vi "Day Total Entries.vi"(8 "error in":errorcluster, 10 "Day":timestamp, 11 "Time Entry Store in":refnum<class "Time Entry Store.lvclass">) -> (0 "error out":errorcluster, 2 "Total Entries":T1, 3 "Time Entry Store out":refnum<class "Time Entry Store.lvclass">)   [LabVIEW 2026]
doc: "Collects the time entries that count towards the total of one local calendar day, for Day Total.vi. Call it once when a day is loaded; it reads the store.\n\nReturns every entry that starts on the day (as the Time Entry Store's Read Entries for Day gives them) plus every entry that started on the previous day and either ends after the day's local midnight or is still running (End Time 0). The previous day is read through the store too, so the store picks the month files (the previous day may be in the previous month). Day starts are calendar-correct local midnights (Increment_Decrement by one Day.vi), so daylight saving days are handled. Entries are de-duplicated by ID and ordered by Start Time.\n\nInputs: Time Entry Store in; Day (any time within the local day); error in.\nOutputs: Time Entry Store out; Total Entries; error out.\n\nGenerated by: Claude"
uses:
  Storage/Time Entry Store/Time Entry Store.lvclass
  Storage/Rows/Time Entry List.ctl
  Storage/Rows/Time Entry.ctl
  Utilities/Time Management/ENUM-Inc_Dec.ctl
  Utilities/Time Management/Time Management.lvlib
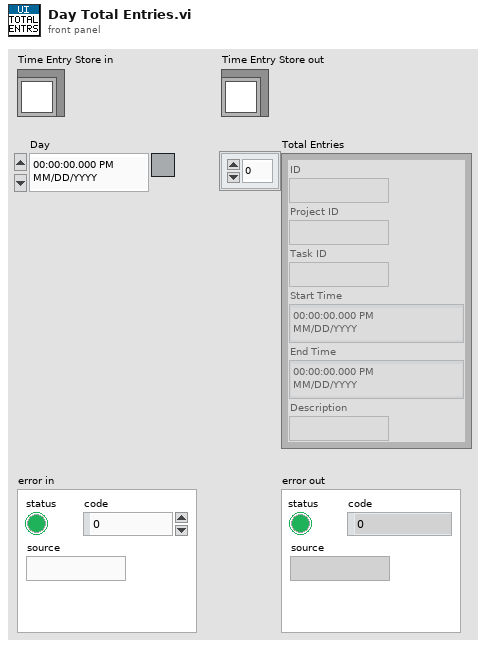
[diagram p1: front panel]
types:
  T1 = typedef "Time Entry List.ctl" = T2[]
  T2 = typedef "Time Entry.ctl" = cluster{"ID":string, "Project ID":string, "Task ID":string, "Start Time":timestamp, "End Time":timestamp, "Description":string}
  T3 = typedef "ENUM-Inc_Dec.ctl" = enum16{"NO CHANGE", "Increment", "Decrement"}
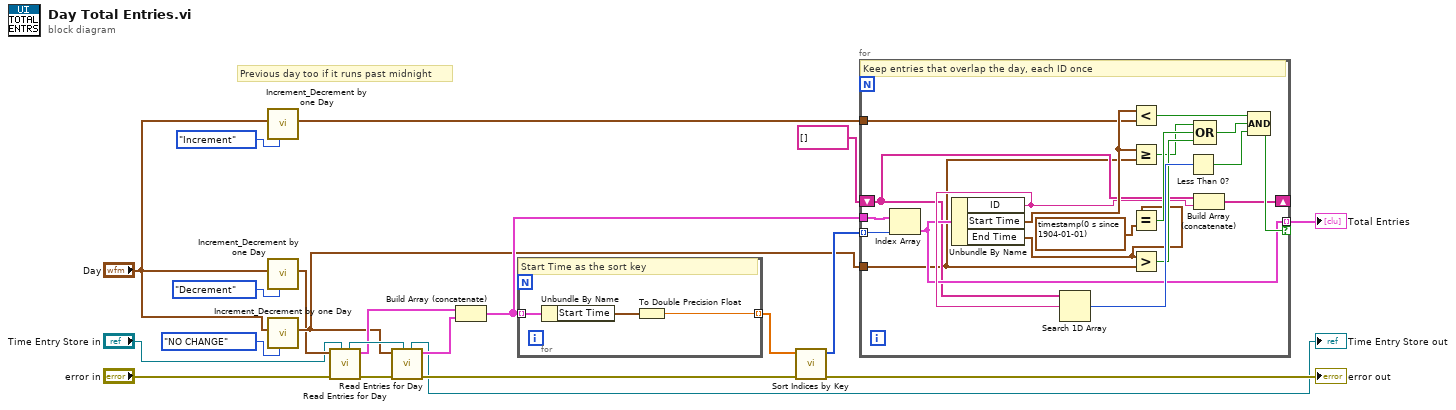
[diagram p0: block diagram]
diagram:
  # "Previous day too if it runs past midnight"
  n1 = call "Increment_Decrement by one Day.vi"("Inc/Dec (No Change)"=ENUM-Inc_Dec."Increment" ("Inc/Dec next day"), "Start Day"="Day") -> ("End Day"=w13:timestamp)  [unwired: 8 in, 1 out]
  n2 = call "Increment_Decrement by one Day.vi"("Inc/Dec (No Change)"=ENUM-Inc_Dec."Decrement" ("Inc/Dec previous day"), "Start Day"="Day") -> ("End Day"=w11:timestamp)  [unwired: 8 in, 1 out]
  n3 = call "Increment_Decrement by one Day.vi"("Inc/Dec (No Change)"=ENUM-Inc_Dec."NO CHANGE" ("Inc/Dec same day"), "Start Day"="Day") -> ("End Day"=w12:timestamp)  [unwired: 8 in, 1 out]
  n4 = call-dynamic "Read Entries for Day.vi"("Time Entry Store in"="Time Entry Store in", "error in (no error)"="error in", "Date"=w11) -> ("error out"=w14:errorcluster, "Time Entries"=w15:T1, "Time Entry Store out"=w16:refnum<class "Time Entry Store.lvclass">)  [unwired: 6 in]
  n5 = call-dynamic "Read Entries for Day.vi"("Time Entry Store in"=w16, "error in (no error)"=w14, "Date"=w12) -> ("error out"=w17:errorcluster, "Time Entries"=w18:T1, "Time Entry Store out"=→"Time Entry Store out":refnum<class "Time Entry Store.lvclass">)  [unwired: 6 in]
  n6 = Build Array (concatenate)(w15, w18) -> (w19:T1)
  n7 = for {
    tunnel: w19 -> [w22] mode=indexing
    tunnel: [w24] -> w20 mode=indexing
    # "Start Time as the sort key"
    n8 = Unbundle By Name(w22) -> ("Start Time"=w23:timestamp)
    n9 = To Double Precision Float(number=w23) -> (double precision float=w24:dbl)
  }
  n10 = call "Sort Indices by Key.vi"("error in (no error)"=w17, "Keys"=w20) -> ("error out"=→"error out":errorcluster, "Sorted Indices"=w21:i32[])  [unwired: 8 in]
  n11 = for {
    shift-right: [w30] -> _
    shift-left: string[] [] ("no IDs yet") -> [w29]
    tunnel: w12 -> [w27]
    tunnel: w13 -> [w28]
    tunnel: w19 -> [w26]
    tunnel: w21 -> [w25] mode=indexing
    tunnel: [w32] -> w5 mode=indexing if=w43
    # "Keep entries that overlap the day, each ID once"
    n12 = Index Array(array=w26, index=w25) -> (element=w32:T2)
    n13 = Unbundle By Name(w32) -> ("ID"=w33:string, "Start Time"=w34:timestamp, "End Time"=w35:timestamp)
    n14 = Search 1D Array(1D array=w29, element=w33) -> (index of element=w41:i32)  [unwired: 1 in]
    n15 = Less?(x=w34, y=w28) -> (x < y?=w36:bool)
    n16 = Greater Or Equal?(x=w34, y=w27) -> (x >= y?=w37:bool)
    n17 = Equal?(x=w35, y=timestamp(0 s since 1904-01-01) ("running End Time")) -> (x = y?=w38:bool)
    n18 = Greater?(x=w35, y=w27) -> (0:w39:bool)
    n19 = Less Than 0?(x=w41) -> (x < 0?=w42:bool)
    n20 = Compound Arithmetic op=OR(w37, w38, w39) -> (w40:bool)
    n21 = Build Array (concatenate)(w29, w33) -> (w30:string[])
    n22 = Compound Arithmetic op=AND(w36, w40, w42) -> (w43:bool)
  }
  "Total Entries" <- w5
